vi "Set Task Active.vi"(7 "Project Store in":refnum<class "Project Store.lvclass">, 8 "error in":errorcluster, 10 "Active?":bool=TRUE, 11 "Task ID":string) -> (0 "error out":errorcluster, 5 "Project Store out":refnum<class "Project Store.lvclass">)   [LabVIEW 2026]
doc: "Makes one task active or inactive and writes the change to the data source, so it survives a restart. Get Task by ID, set Active, Update Task, Write to Data Source. An unknown Task ID changes nothing (the data source is still rewritten unchanged).\n\nInputs: Task ID; Active?; Project Store in; error in.\nOutputs: Project Store out; error out.\n\nGenerated by: Claude"
uses:
  Storage/Project Store/Project Store.lvclass
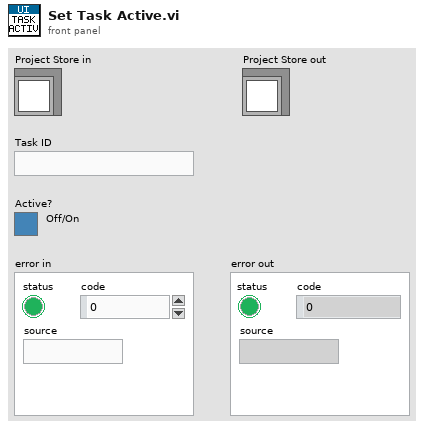
[diagram p1: front panel]
types:
  T1 = typedef "Task.ctl" = cluster{"ID":string, "Project ID":string, "Name":string, "Active":bool, "Sort Order":i32}
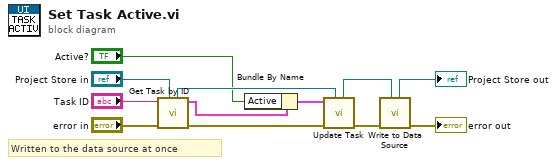
[diagram p0: block diagram]
diagram:
  # "Written to the data source at once"
  n1 = call-dynamic "Get Task by ID.vi"("Project Store in"="Project Store in", "error in (no error)"="error in", "ID"="Task ID") -> ("error out"=w9:errorcluster, "Task"=w7:T1, "Project Store out"=w8:refnum<class "Project Store.lvclass">)  [unwired: 5 in, 1 out]
  n2 = Bundle By Name(cluster=w7, "Active"="Active?") -> (w10:T1)
  n3 = call-dynamic "Update Task.vi"("Project Store in"=w8, "error in (no error)"=w9, "Task"=w10) -> ("error out"=w12:errorcluster, "Project Store out"=w11:refnum<class "Project Store.lvclass">)  [unwired: 6 in, 1 out]
  n4 = call-dynamic "Write to Data Source.vi"("Project Store in"=w11, "error in (no error)"=w12) -> ("error out"=→"error out":errorcluster, "Project Store out"=→"Project Store out":refnum<class "Project Store.lvclass">)  [unwired: 8 in]
